vi "Tool List Cache.vi"(7 "write? (F)":bool, 8 "error in":errorcluster, 9 "tools json":string, 10 "key":string, 11 "server id":i32) -> (0 "error out":errorcluster, 2 "tools json out":string, 3 "found?":bool)   [LabVIEW 2020, in "MCP Server.lvlib"]
doc: "Keeps the built result of tools/list per MCP server, so that Cached Tool List.vi does not build it again for every request. A functional global (not reentrant): the entries live in the shift registers of this VI.\n\nEach entry is the server id, a key and the result JSON ({\"tools\":[...]}). The key is the flattened Tools array of the server at the time the list was built. An entry is only returned for the same key, so a list built for other tools is never returned: after Add Tool.vi or Clear Tools.vi the key differs and the caller builds the list again. No VI has to invalidate the cache.\n\nwrite? FALSE (default): looks up server id. found? is TRUE and tools json out is the stored result when there is an entry for server id whose key equals key.\nwrite? TRUE: stores key and tools json for server id, replacing the entry of that server. found? is FALSE and tools json out is tools json.\n\nAt most 16 servers are kept: when a 17th is stored all entries are dropped first, so entries of servers that were stopped do not pile up. error in is passed to error out and does not change what the VI does."
uses:
  MCP Server.lvlib
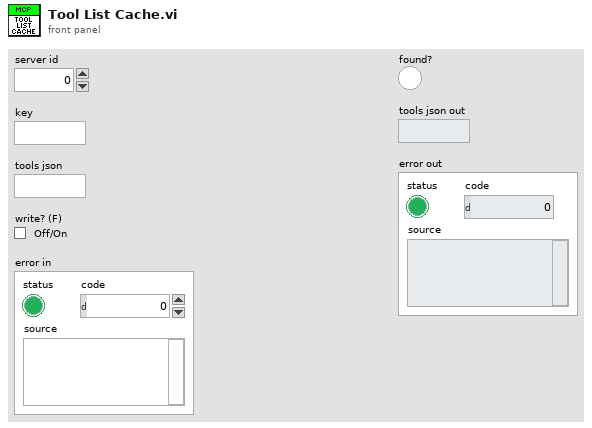
[diagram p1: front panel]
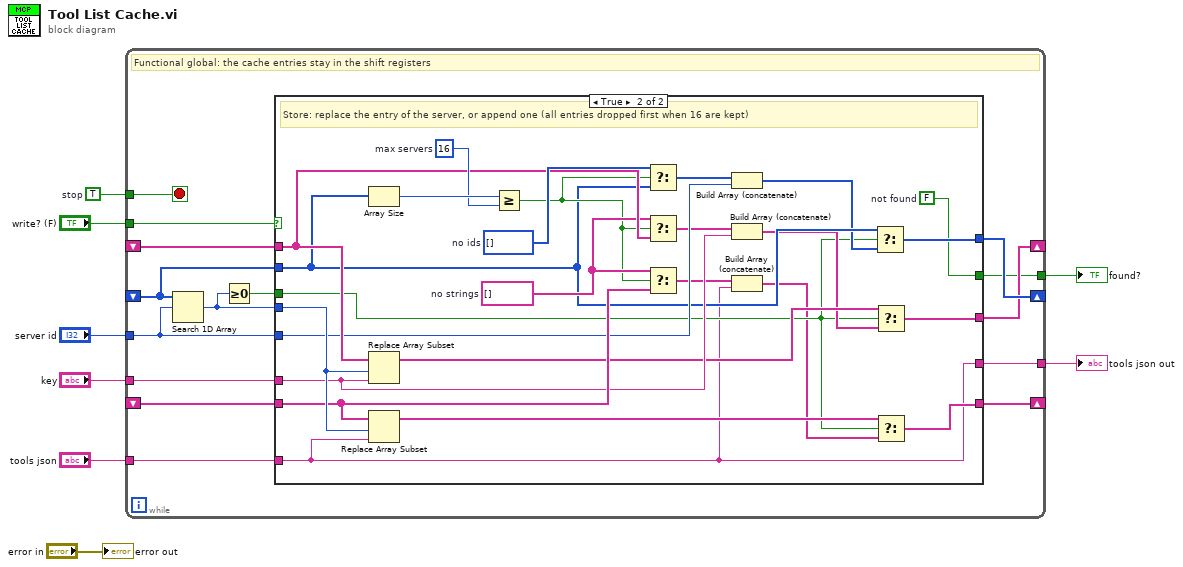
[diagram p0: block diagram]
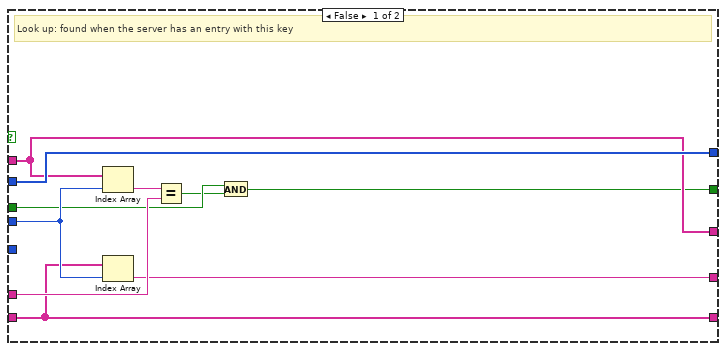
[diagram p2: hidden frame]
diagram:
  w4 = TRUE  # stop
  n1 = while {
    tunnel: "server id" -> [w17]
    tunnel: "key" -> [w16]
    tunnel: "tools json" -> [w15]
    tunnel: "write? (F)" -> [w11]
    tunnel: w4 -> [w23]
    shift-right: [w14] -> _
    shift-left: _ -> [w22]
    shift-right: [w13] -> _
    shift-left: _ -> [w21]
    shift-right: [w12] -> _
    shift-left: _ -> [w20]
    tunnel: [w10] -> w3
    tunnel: [w9] -> w2
    stop <- w23 stop-if-true
    # "Functional global: the cache entries stay in the shift registers"
    n2 = Search 1D Array(1D array=w22, element=w17) -> (index of element=w19:i32)  [unwired: 1 in]
    n3 = Greater Or Equal To 0?(x=w19) -> (x >= 0?=w18:bool)
    n4 = case shown="True" w11 {
      tunnel: w22 -> [w28 w45]
      tunnel: w21 -> [w27 w54]
      tunnel: w20 -> [w26 w51]
      tunnel: w19 -> [w33 w58]
      tunnel: w18 -> [w30 w40]
      tunnel: w17 -> [_ w49]
      tunnel: w16 -> [w31 w47]
      tunnel: w15 -> [_ w34]
      tunnel: [w28 w38] -> w14
      tunnel: [w27 w37] -> w13
      tunnel: [w26 w36] -> w12
      tunnel: [w25 w35] -> w10
      tunnel: [w24 w34] -> w9
      frame False {
        # "Look up: found when the server has an entry with this key"
        n5 = Index Array(array=w27, index=w33) -> (element=w32:string)
        n6 = Index Array(array=w26, index=w33) -> (element=w24:string)
        n7 = Equal?(x=w32, y=w31) -> (x = y?=w29:bool)
        n8 = And(x=w30, y=w29) -> (x .and. y?=w25:bool)
      }
      frame True {
        w35 = FALSE  # not found
        w53 = string[] []  # no strings
        w55 = i32[] []  # no ids
        w56 = 16  # max servers
        # "Store: replace the entry of the server, or append one (all entries dropped first when 16 are kept)"
        n9 = Array Size(array=w45) -> (size(s)=w57:i32)
        n10 = Replace Array Subset(array=w54, new element=w47, index=w58) -> (w43:string[])
        n11 = Replace Array Subset(array=w51, new element=w34, index=w58) -> (w41:string[])
        n12 = Greater Or Equal?(x=w57, y=w56) -> (x >= y?=w52:bool)
        n13 = Select(t=w55, s=w52, f=w45) -> (s? t:f=w50:i32[])
        n14 = Select(t=w53, s=w52, f=w54) -> (s? t:f=w48:string[])
        n15 = Select(t=w53, s=w52, f=w51) -> (s? t:f=w46:string[])
        n16 = Build Array (concatenate)(w50, w49) -> (w44:i32[])
        n17 = Build Array (concatenate)(w48, w47) -> (w42:string[])
        n18 = Build Array (concatenate)(w46, w34) -> (w39:string[])
        n19 = Select(t=w45, s=w40, f=w44) -> (s? t:f=w38:i32[])
        n20 = Select(t=w43, s=w40, f=w42) -> (s? t:f=w37:string[])
        n21 = Select(t=w41, s=w40, f=w39) -> (s? t:f=w36:string[])
      }
    }
  }
  "found?" <- w3
  "tools json out" <- w2
  "error out" <- "error in"
